vi "Main.vi"(11 "Error In":errorcluster) -> (15 "Error Out":errorcluster)   [LabVIEW 2026]
uses:
  Core/TypeDefs/Enum_Events.ctl
  Core/TypeDefs/Enum_Event_Options.ctl
  Core/TypeDefs/Enum_Queue_Options.ctl
  Core/TypeDefs/Cluster_Queue_Element.ctl
  Core/TypeDefs/Enum_Queues.ctl
  Core/SubVIs/Status_Page/INL-DNL-Status.vi
  Core/Core.lvlib
panel:
  out "Status & Graph":picture
  out "Configuration":picture
  out "Mode Selection":picture
  out "Home":picture
  in  "Tab Sel Buttons":T1(radio)
  in  "Tab Control":T1(tab)
  out "DAC":picture
  out "ADC":picture
  out "Mode Sel Buttons":enum32{"ADC", "DAC"}(radio)
  out "Configuration String":string
  out "Status & Graph String":string
  out "Status":string[][](table)
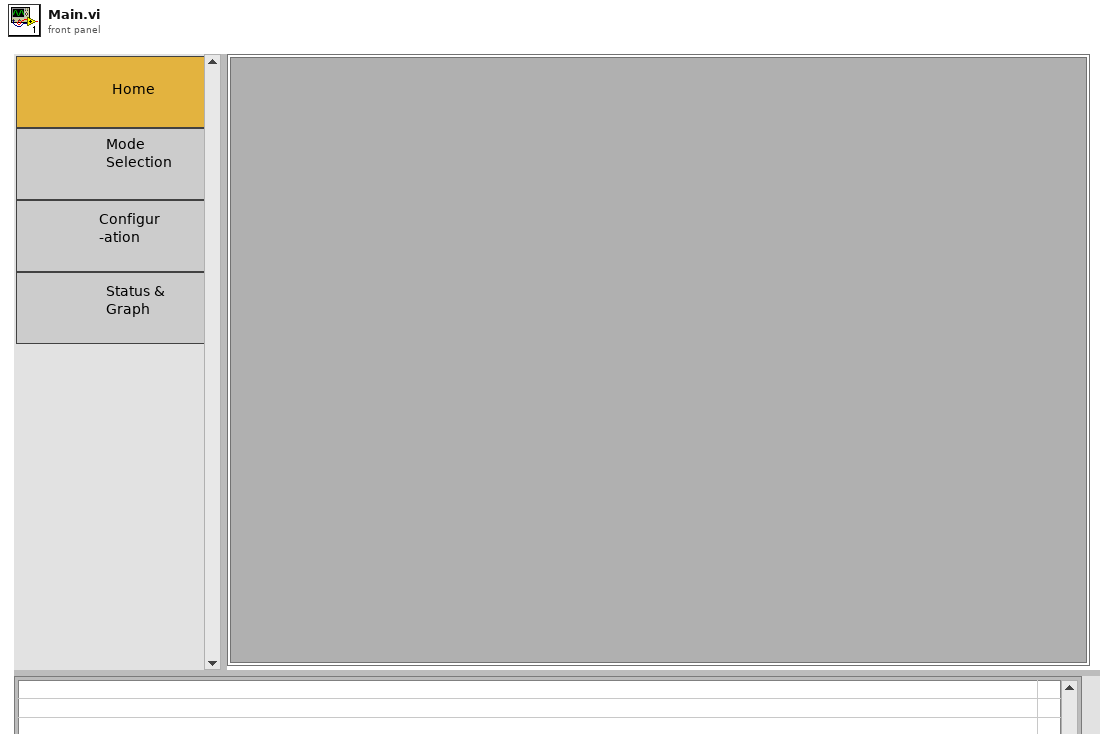
[diagram p1: front panel]
types:
  T1 = enum32{"Home", "Mode Selection", "Configuration", "Status & Graph"}
  T2 = typedef "Core.lvlib/Cluster_Queue_Element.ctl" = cluster{"State":string, "Data":variant}
  T3 = typedef "Core.lvlib/Enum_Queue_Options.ctl" = enum16{"Create", "Enqueue N", "Enstack N", "View Queue", "Dequeue", "Flush", "Flush & Close"}
  T4 = typedef "Core.lvlib/Enum_Queues.ctl" = enum16{"State"}
  T5 = typedef "Core.lvlib/Enum_Event_Options.ctl" = enum16{"Create", "Generate", "Event Ref", "Destroy"}
  T6 = typedef "Core.lvlib/Enum_Events.ctl" = enum16{"Stop All", "Stop SubVI", "Update Object"}
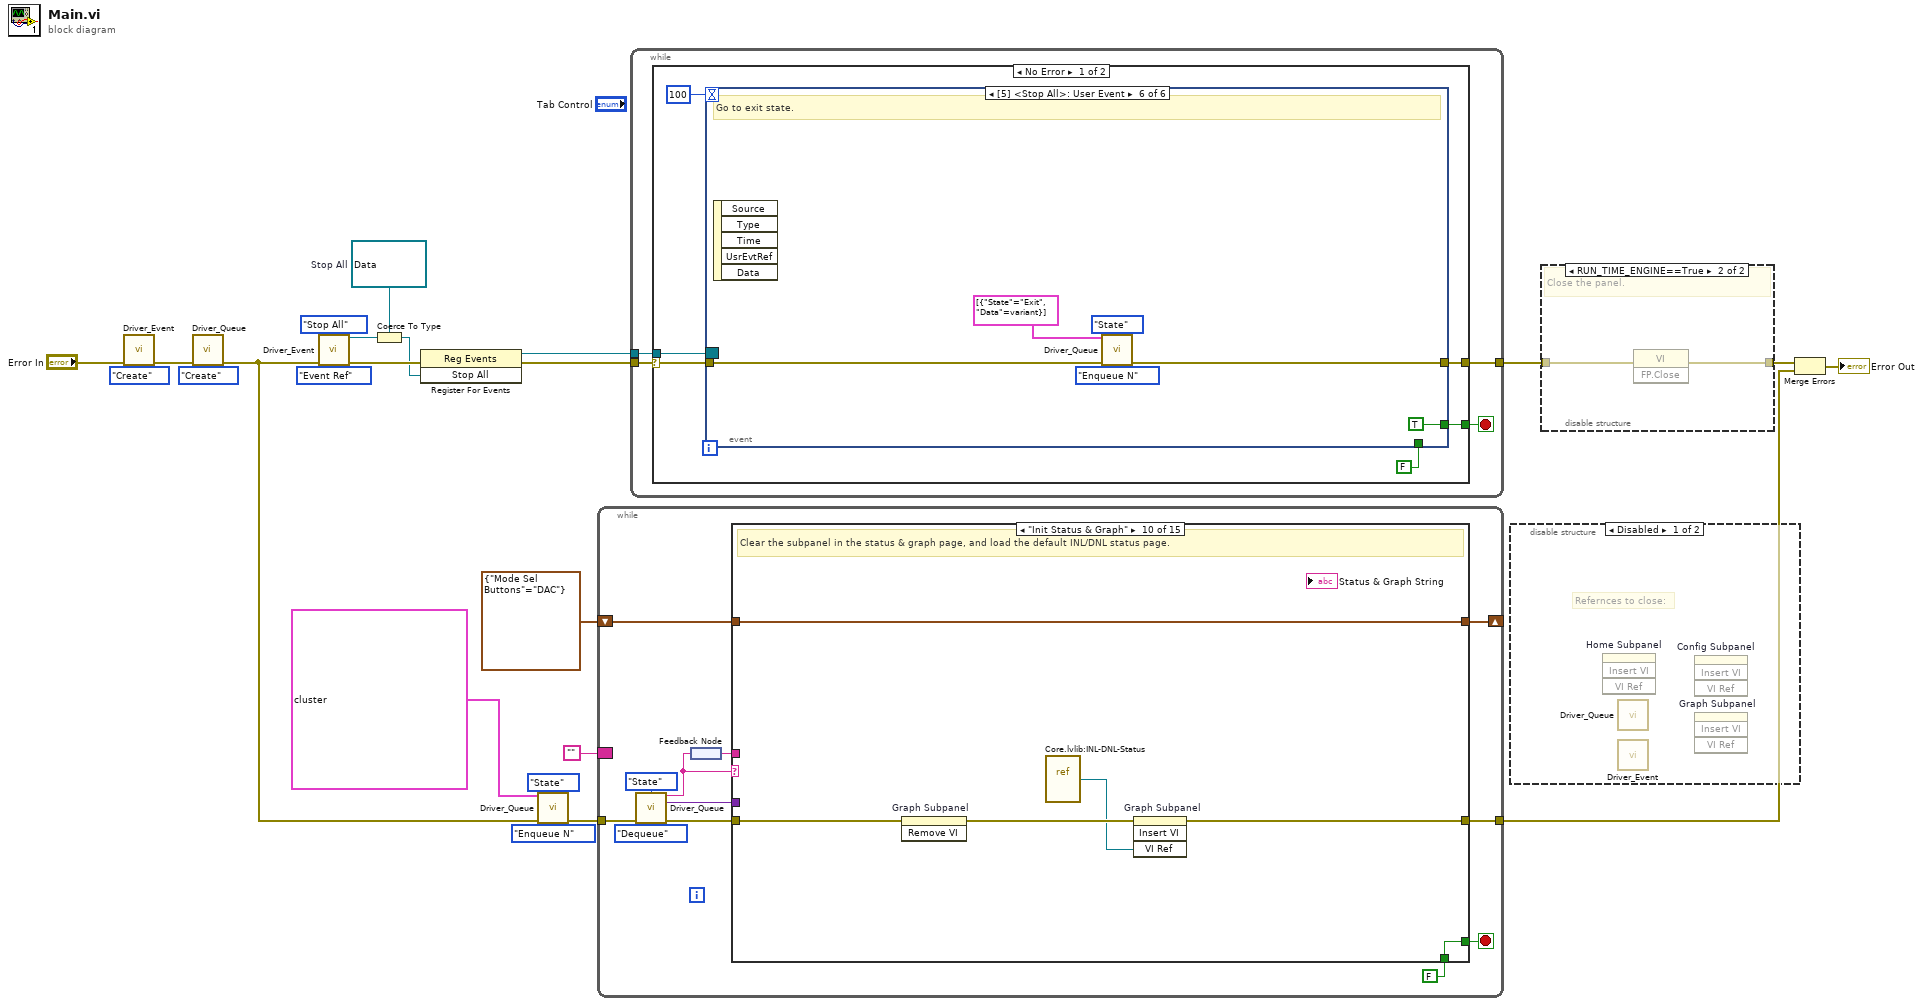
[diagram p0: block diagram]
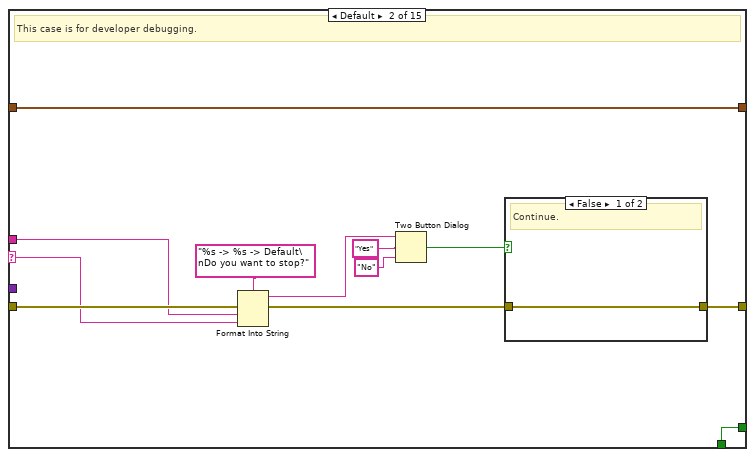
[diagram p5: hidden frame]
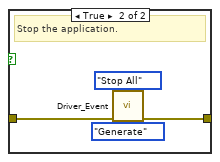
[diagram p6: hidden frame]
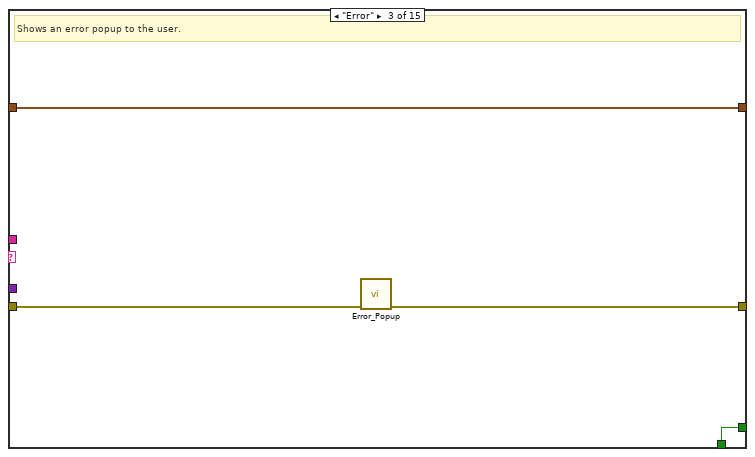
[diagram p7: hidden frame]
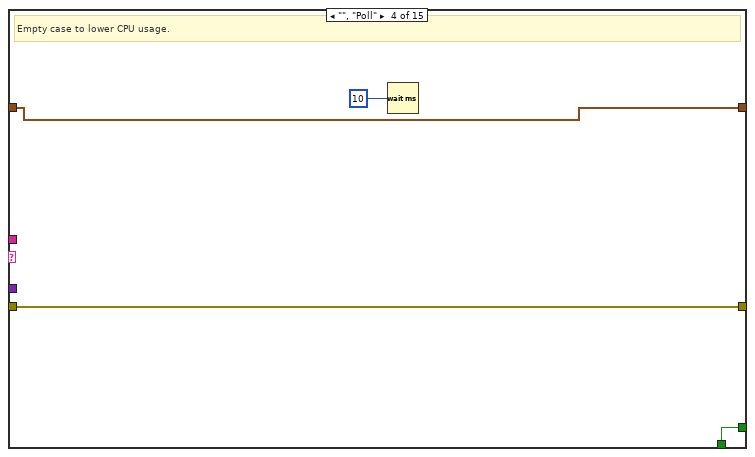
[diagram p8: hidden frame]
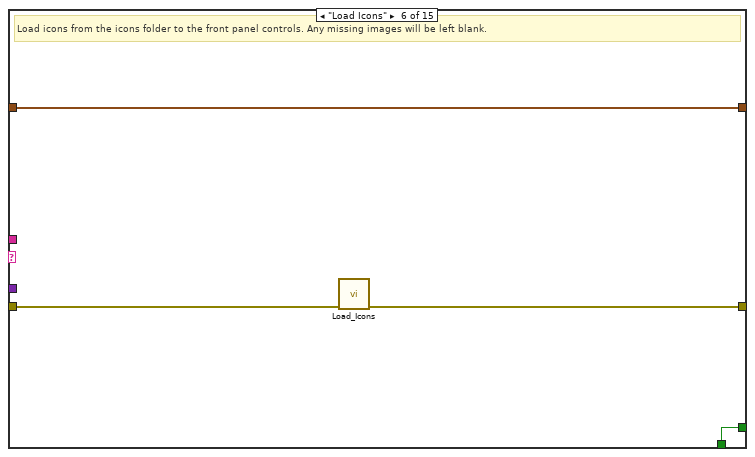
[diagram p10: hidden frame]
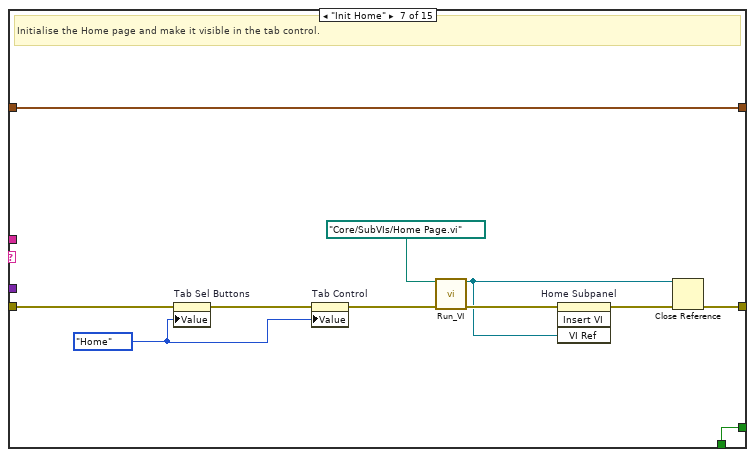
[diagram p11: hidden frame]
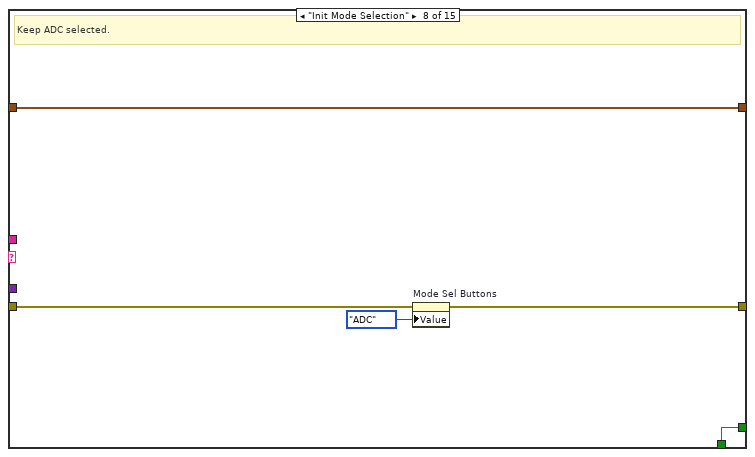
[diagram p12: hidden frame]
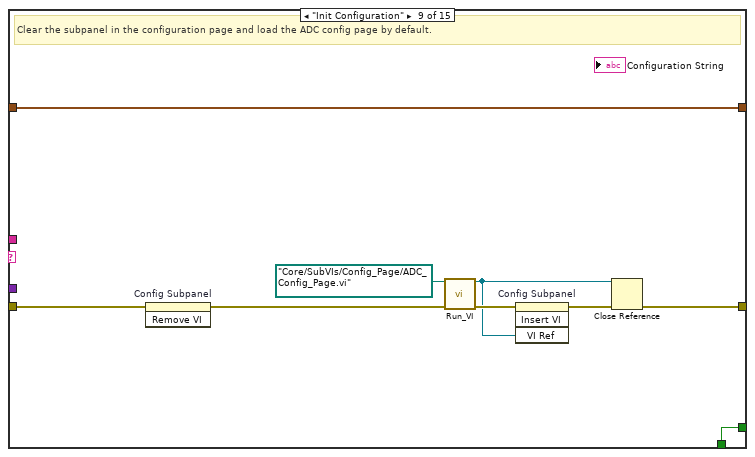
[diagram p13: hidden frame]
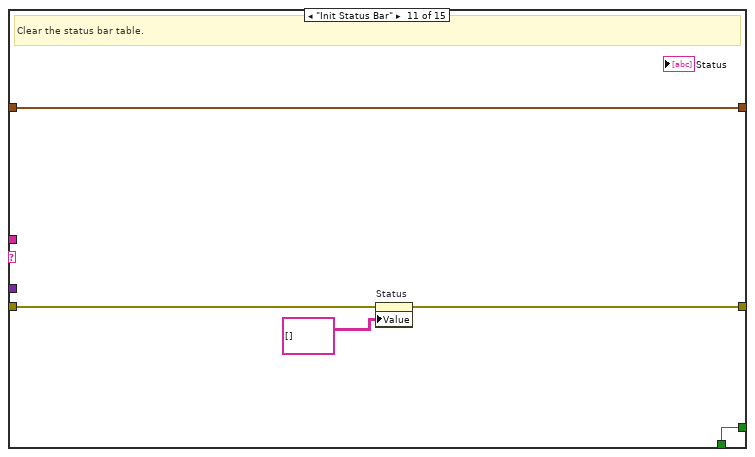
[diagram p14: hidden frame]
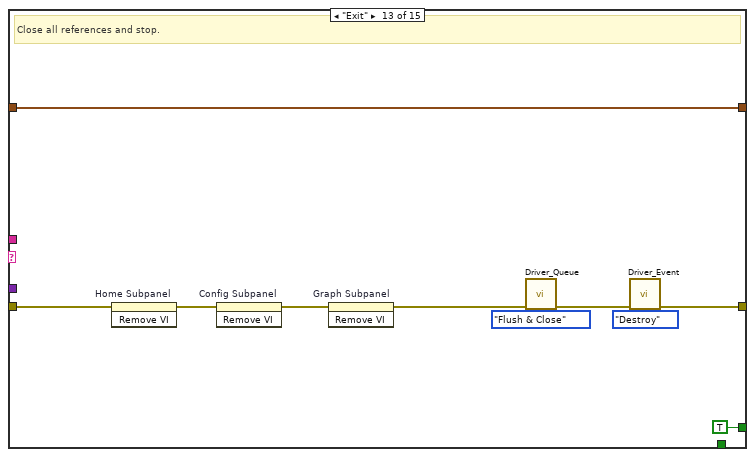
[diagram p16: hidden frame]
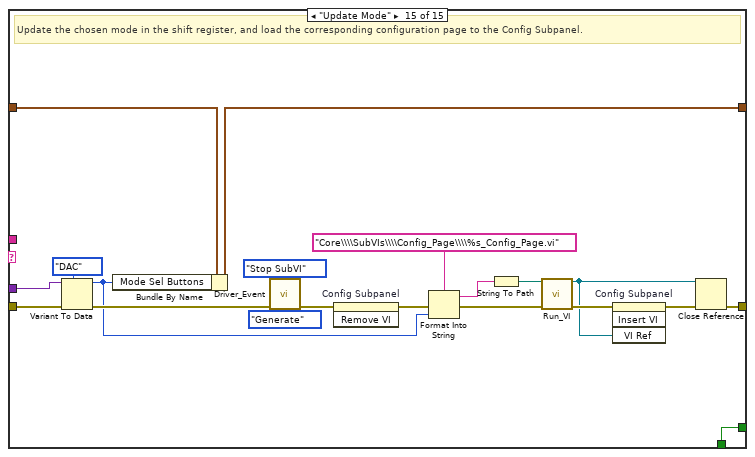
[diagram p18: hidden frame]
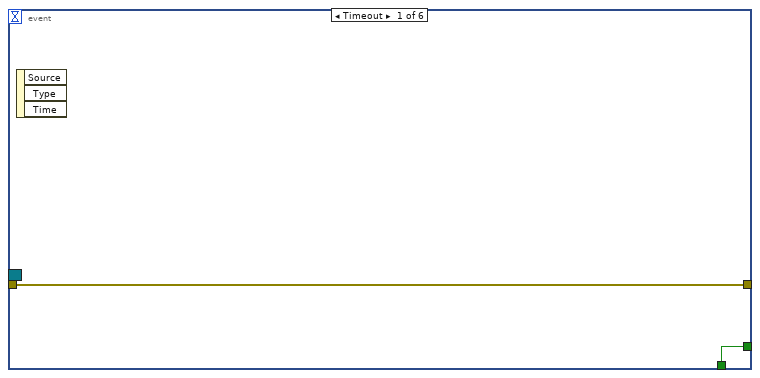
[diagram p19: hidden frame]
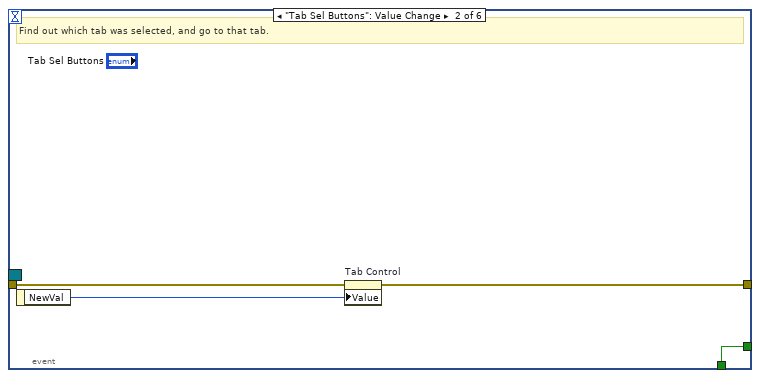
[diagram p20: hidden frame]
diagram:
  w17 = refnum<user-event> refnum  # Stop All
  n1 = call "Driver_Event.vi"("Error In"="Error In", "Event Operation"=Enum_Event_Options."Create") -> ("Error Out"=w22:errorcluster)  [unwired: 12 in, 1 out]
  n2 = call "Driver_Queue.vi"("Error In"=w22, "Queue Operation"=Enum_Queue_Options."Create") -> ("Error Out"=w11:errorcluster)  [unwired: 10 in, 3 out]
  n3 = call "Driver_Event.vi"("Event"=Enum_Events."Stop All", "Error In"=w11, "Event Operation"=Enum_Event_Options."Event Ref") -> ("Event Ref"=w20:refnum<user-event>, "Error Out"=w19:errorcluster)  [unwired: 11 in]
  n4 = Coerce To Type(0:w20, 1:w17) -> (2:w18:refnum<user-event>)
  n5 = register-events(error in=w19, w18) -> (reference out=w12:refnum<event-registration>, error out=w21:errorcluster)  [unwired: 1 in]
  n6 = call "Driver_Queue.vi"("Queue N Elements"=T2[] [{"State"="Load Icons", "Data"=variant}, {"State"="Init Home", "Data"=variant}, {"State"="Init Mode Selection", "Data"=variant}, {"State"="Init Configuration", "Data"=variant}, {"State"="Init Status & Graph", "Data"=variant}, {"State"="Init Status Bar", "Data"=variant}], "Queue"=Enum_Queues."State", "Error In"=w11, "Queue Operation"=Enum_Queue_Options."Enqueue N") -> ("Error Out"=w10:errorcluster)  [unwired: 8 in, 3 out]
  n7 = while {
    tunnel: w10 -> [w32]
    tunnel: [w35] -> w2
    border: "" -> [_]
    shift-right: [w24] -> _
    shift-left: cluster{"Mode Sel Buttons":enum32{"ADC", "DAC"}} {"Mode Sel Buttons"=enum."DAC"} -> [w25]
    stop <- w34 stop-if-true
    n8 = call "Driver_Queue.vi"("Queue"=Enum_Queues."State", "Error In"=w32, "Queue Operation"=Enum_Queue_Options."Dequeue") -> ("State"=w27:string, "Data"=w28:variant, "Error Out"=w31:errorcluster)  [unwired: 9 in, 1 out]
    n9 = feedback-in #1(w27) -> ()
    n10 = feedback #1() -> (w26:string)
    n11 = case shown="\"Init Status & Graph\"" w27 {
      selector: w27 -> [_ w47 _ _ _ _ _ _ _ _ _ _ _ _ _]
      tunnel: [w38 w42 w58 w62 w66 w69 w77 w83 w88 w97 w105 w109 w114 w122 w124] -> w35
      tunnel: [w37 w40 w57 w61 w65 w68 w80 w86 w94 w100 w104 w108 TRUE w121 w137] -> w34
      tunnel: FALSE -> [w37 w40 w57 w61 w65 w68 w80 w86 w94 w100 w104 w108 _ w121 w137]
      tunnel: w31 -> [w38 w50 w59 w62 w66 w70 w74 w84 w95 w101 w106 w109 w119 w122 w142]
      tunnel: w28 -> [_ _ _ _ _ _ _ _ _ _ _ _ _ _ w141]
      tunnel: w26 -> [_ w48 _ _ _ _ _ _ _ _ _ _ _ _ _]
      tunnel: w25 -> [w36 w39 w56 w60 w64 w67 w71 w85 w93 w99 w102 w107 w110 w120 w139]
      tunnel: [w36 w39 w56 w60 w64 w67 w71 w85 w93 w99 w102 w107 w110 w120 w138] -> w24
      frame "/-----General-----/" {
      }
      frame Default {
        # "This case is for developer debugging."
        n12 = Format Into String(format string="%s -> %s -> Default\nDo you want to stop?", error in=w50, w48, w47) -> (resulting string=w46:string, error out=w43:errorcluster)  [unwired: 1 in]
        n13 = Two Button Dialog(message=w46, 1:"No" ("F button name (\"Cancel\")"), 2:"Yes" ("T button name (\"OK\")")) -> (T button?=w41:bool)
        n14 = case shown="False" w41 {
          tunnel: w43 -> [w51 w55]
          tunnel: [w51 w54] -> w42
          frame False {
            # "Continue."
          }
          frame True {
            # "Stop the application."
            n15 = call "Driver_Event.vi"("Event"=Enum_Events."Stop All", "Error In"=w55, "Event Operation"=Enum_Event_Options."Generate") -> ("Error Out"=w54:errorcluster)  [unwired: 11 in, 1 out]
          }
        }
      }
      frame "Error" {
        # "Shows an error popup to the user."
        n16 = call "Error_Popup.vi"("Error In"=w59) -> ("Error Out"=w58:errorcluster)  [unwired: 13 in, 1 out]
      }
      frame "", "Poll" {
        # "Empty case to lower CPU usage."
        n17 = Wait (ms)(milliseconds to wait=u32 10) -> ()  [unwired: 1 out]
      }
      frame "/-----Initialisation-----/" {
      }
      frame "Load Icons" {
        # "Load icons from the icons folder to the front panel controls. Any missing images will be left blank."
        n18 = call "Load_Icons.vi"("Error In"=w70) -> ("Error Out"=w69:errorcluster)  [unwired: 14 in]
      }
      frame "Init Home" {
        w72 = T1."Home" ("Tab Control")
        # "Initialise the Home page and make it visible in the tab control."
        n19 = property on="Tab Sel Buttons" class="RadioBtnsControl (strict)"(error in=w74, "Value"=w72) -> (error out=w73:errorcluster)  [unwired: 1 in, 1 out]
        n20 = property on="Tab Control" class="TabCtl (strict)"(error in=w73, "Value"=w72) -> (error out=w75:errorcluster)  [unwired: 1 in, 1 out]
        n21 = call "Run_VI.vi"("Path"=path "Core/SubVIs/Home Page.vi", "Error In"=w75) -> ("VI Refnum"=w76:refnum<vi>, "Error Out"=w79:errorcluster)  [unwired: 12 in]
        n22 = invoke on="Home Subpanel" class="SubPnl" method="Insert VI"(error in=w79, "VI Ref"=w76) -> (error out=w81:errorcluster)  [unwired: 2 in, 3 out]
        n23 = Close Reference(reference=w76, error in (no error)=w81) -> (error out=w77:errorcluster)
      }
      frame "Init Mode Selection" {
        # "Keep ADC selected."
        n24 = property on="Mode Sel Buttons" class="RadioBtnsControl (strict)"(error in=w84, "Value"=enum32{"ADC", "DAC"}."ADC" ("Mode Sel Buttons")) -> (error out=w83:errorcluster)  [unwired: 1 in, 1 out]
      }
      frame "Init Configuration" {
        # "Clear the subpanel in the configuration page and load the ADC config page by default."
        n25 = invoke on="Config Subpanel" class="SubPnl" method="Remove VI"(error in=w95) -> (error out=w91:errorcluster)  [unwired: 2 in, 2 out]
        n26 = call "Run_VI.vi"("Path"=path "Core/SubVIs/Config_Page/ADC_Config_Page.vi", "Error In"=w91) -> ("VI Refnum"=w87:refnum<vi>, "Error Out"=w92:errorcluster)  [unwired: 12 in]
        n27 = invoke on="Config Subpanel" class="SubPnl" method="Insert VI"(error in=w92, "VI Ref"=w87) -> (error out=w90:errorcluster)  [unwired: 2 in, 3 out]
        n28 = Close Reference(reference=w87, error in (no error)=w90) -> (error out=w88:errorcluster)
      }
      frame "Init Status & Graph" {
        # "Clear the subpanel in the status & graph page, and load the default INL/DNL status page."
        n29 = invoke on="Graph Subpanel" class="SubPnl" method="Remove VI"(error in=w101) -> (error out=w98:errorcluster)  [unwired: 2 in, 2 out]
        n30 = vi-ref "Core.lvlib:INL-DNL-Status.vi"() -> (w96:refnum<vi>)
        n31 = invoke on="Graph Subpanel" class="SubPnl" method="Insert VI"(error in=w98, "VI Ref"=w96) -> (error out=w97:errorcluster)  [unwired: 2 in, 3 out]
      }
      frame "Init Status Bar" {
        # "Clear the status bar table."
        n32 = property on="Status" class="Tbl (strict)"(error in=w106, "Value"=string[][] [] ("Status")) -> (error out=w105:errorcluster)  [unwired: 1 in, 1 out]
      }
      frame "/-----Exit-----/" {
      }
      frame "Exit" {
        # "Close all references and stop."
        n33 = invoke on="Home Subpanel" class="SubPnl" method="Remove VI"(error in=w119) -> (error out=w118:errorcluster)  [unwired: 2 in, 2 out]
        n34 = invoke on="Config Subpanel" class="SubPnl" method="Remove VI"(error in=w118) -> (error out=w117:errorcluster)  [unwired: 2 in, 2 out]
        n35 = invoke on="Graph Subpanel" class="SubPnl" method="Remove VI"(error in=w117) -> (error out=w116:errorcluster)  [unwired: 2 in, 2 out]
        n36 = call "Driver_Queue.vi"("Error In"=w116, "Queue Operation"=Enum_Queue_Options."Flush & Close") -> ("Error Out"=w115:errorcluster)  [unwired: 10 in, 3 out]
        n37 = call "Driver_Event.vi"("Error In"=w115, "Event Operation"=Enum_Event_Options."Destroy") -> ("Error Out"=w114:errorcluster)  [unwired: 12 in, 1 out]
      }
      frame "/-----Mode Selection-----/" {
      }
      frame "Update Mode" {
        # "Update the chosen mode in the shift register, and load the corresponding configuration page to the Config Subpanel."
        n38 = Variant To Data(error in=w142, type=enum32{"ADC", "DAC"}."DAC" ("Mode Sel Buttons"), Variant=w141) -> (data=w131:enum32{"ADC", "DAC"}, error out=w136:errorcluster)
        n39 = Bundle By Name(cluster=w139, "Mode Sel Buttons"=w131) -> (w138:cluster{"Mode Sel Buttons":enum32{"ADC", "DAC"}})
        n40 = call "Driver_Event.vi"("Event"=Enum_Events."Stop SubVI", "Error In"=w136, "Event Operation"=Enum_Event_Options."Generate") -> ("Error Out"=w126:errorcluster)  [unwired: 11 in, 1 out]
        n41 = invoke on="Config Subpanel" class="SubPnl" method="Remove VI"(error in=w126) -> (error out=w125:errorcluster)  [unwired: 2 in, 2 out]
        n42 = Format Into String(format string="Core\\\\SubVIs\\\\Config_Page\\\\%s_Config_Page.vi", error in=w125, w131) -> (resulting string=w130:string, error out=w133:errorcluster)  [unwired: 1 in]
        n43 = String To Path(string=w130) -> (path=w129:path)
        n44 = call "Run_VI.vi"("Path"=w129, "Error In"=w133) -> ("VI Refnum"=w123:refnum<vi>, "Error Out"=w128:errorcluster)  [unwired: 12 in]
        n45 = invoke on="Config Subpanel" class="SubPnl" method="Insert VI"(error in=w128, "VI Ref"=w123) -> (error out=w127:errorcluster)  [unwired: 2 in, 3 out]
        n46 = Close Reference(reference=w123, error in (no error)=w127) -> (error out=w124:errorcluster)
      }
    }
  }
  n47 = while {
    tunnel: w21 -> [w146]
    tunnel: [w145] -> w5
    tunnel: w12 -> [w144]
    stop <- w143 stop-if-true
    n48 = case shown="No Error" w146 {
      selector: w146 -> [w151 w214]
      tunnel: [w150 w213] -> w145
      tunnel: w144 -> [w149 _]
      tunnel: [w148 FALSE] -> w143
      frame No Error {
        n49 = event shown="[5] <Stop All>: User Event" {
          selector: w149 -> [_ _ _ _ _ _]
          dyn-events: _ -> [_ _ _ _ _ _]
          timeout: 100 -> [_ _ _ _ _ _]
          tunnel: w151 -> [w154 w156 w167 w192 w205 w211]
          tunnel: [w154 w158 w160 w186 w204 w210] -> w150
          tunnel: [w153 w157 w165 w188 w203 TRUE] -> w148
          tunnel: FALSE -> [w153 w157 w165 w188 w203 _]
          event Timeout {
            n50 = event-data() -> ()  [unwired: 1 in, 3 out]
          }
          event "Tab Sel Buttons": Value Change {
            # "Find out which tab was selected, and go to that tab."
            n51 = event-data() -> ("NewVal"=w155:T1)  [unwired: 1 in]
            n52 = property on="Tab Control" class="TabCtl (strict)"(error in=w156, "Value"=w155) -> (error out=w158:errorcluster)  [unwired: 1 in, 1 out]
          }
          event "Home", "Mode Selection", "Configuration", "Status & Graph": Mouse Down {
            # "Even if the tab images are clicked, the tab should change."
            n53 = event-data() -> ("CtlRef"=w164:refnum<vi>)  [unwired: 1 in]
            n54 = property class="Pict"(reference=w164, error in=w167) -> (error out=w161:errorcluster, "Label.Text"=w163:string)  [unwired: 1 out]
            n55 = case shown="\"Status & Graph\"" w163 {
              tunnel: [T1."Home" ("Tab Control") T1."Home" ("Tab Control") T1."Mode Selection" ("Tab Control") T1."Configuration" ("Tab Control") T1."Status & Graph" ("Tab Control")] -> w159
              tunnel: [w169 w170 w173 w175 w177] -> w162
              tunnel: w161 -> [w169 w170 w173 w175 w177]
              frame Default {
                # "Set Home as default."
              }
              frame "Home" {
                # "Set the tab to Home."
              }
              frame "Mode Selection" {
                # "Set the tab to Mode Selection."
              }
              frame "Configuration" {
                # "Set the tab to Configuration."
              }
              frame "Status & Graph" {
                # "Set the tab to Status & Graph."
              }
            }
            n56 = property on="Tab Control" class="TabCtl (strict)"(error in=w162, "Value"=w159) -> (error out=w166:errorcluster)  [unwired: 1 in, 1 out]
            n57 = property on="Tab Sel Buttons" class="RadioBtnsControl (strict)"(error in=w166, "Value"=w159) -> (error out=w160:errorcluster)  [unwired: 1 in, 1 out]
          }
          event "ADC", "DAC": Mouse Down {
            # "Highlight the selected device."
            n58 = event-data() -> ("CtlRef"=w193:refnum<vi>)  [unwired: 1 in]
            n59 = property class="Pict"(reference=w193, error in=w192) -> (error out=w190:errorcluster, "Label.Text"=w191:string)  [unwired: 1 out]
            n60 = case shown="\"DAC\"" w191 {
              tunnel: [w195 w197 w199] -> w189
              tunnel: w190 -> [w195 w197 w199]
              tunnel: [enum32{"ADC", "DAC"}."ADC" ("Mode Sel Buttons") enum32{"ADC", "DAC"}."ADC" ("Mode Sel Buttons") enum32{"ADC", "DAC"}."DAC" ("Mode Sel Buttons")] -> w180
              frame Default {
                # "Keep ADC as default."
              }
              frame "ADC" {
                # "Make ADC highlighted."
              }
              frame "DAC" {
                # "Make DAC highlighted."
              }
            }
            n61 = property on="Mode Sel Buttons" class="RadioBtnsControl (strict)"(error in=w189, "Value"=w180) -> (error out=w187:errorcluster)  [unwired: 1 in, 1 out]
            n62 = To Variant(anything=w180) -> (Variant=w181:variant)
            n63 = Bundle By Name(cluster=T2 {"State"="", "Data"=variant} ("Queue Element"), "State"="Update Mode", "Data"=w181) -> (w179:T2)
            n64 = Build Array(w179) -> (w178:T2[])
            n65 = call "Driver_Queue.vi"("Queue N Elements"=w178, "Queue"=Enum_Queues."State", "Error In"=w187, "Queue Operation"=Enum_Queue_Options."Enqueue N") -> ("Error Out"=w186:errorcluster)  [unwired: 8 in, 3 out]
          }
          event Panel Close? {
            # "This stops the application."
            n66 = event-data() -> ()  [unwired: 1 in, 1 out]
            n67 = call "Driver_Event.vi"("Event"=Enum_Events."Stop All", "Error In"=w205, "Event Operation"=Enum_Event_Options."Generate") -> ("Error Out"=w204:errorcluster)  [unwired: 11 in, 1 out]
            n68 = event-data("Discard?"=TRUE) -> ()  [unwired: 1 in, 1 out]
          }
          event User Event {
            # "Go to exit state."
            n69 = event-data() -> ()  [unwired: 1 in, 5 out]
            n70 = call "Driver_Queue.vi"("Queue N Elements"=T2[] [{"State"="Exit", "Data"=variant}], "Queue"=Enum_Queues."State", "Error In"=w211, "Queue Operation"=Enum_Queue_Options."Enqueue N") -> ("Error Out"=w210:errorcluster)  [unwired: 8 in, 3 out]
          }
        }
      }
      frame Error {
        n71 = call "Error_Popup.vi"("Error In"=w214) -> ("Error Out"=w213:errorcluster)  [unwired: 13 in, 1 out]
      }
    }
  }
  n72 = disable-structure shown="Disabled" {
    frame Disabled {
      # "Refernces to close:"
      n73 = invoke on="Home Subpanel" class="SubPnl" method="Insert VI"() -> ()  [unwired: 4 in, 4 out]
      n74 = call "Driver_Queue.vi"() -> ()  [unwired: 12 in, 4 out]
      n75 = call "Driver_Event.vi"() -> ()  [unwired: 14 in, 2 out]
      n76 = invoke on="Config Subpanel" class="SubPnl" method="Insert VI"() -> ()  [unwired: 4 in, 4 out]
      n77 = invoke on="Graph Subpanel" class="SubPnl" method="Insert VI"() -> ()  [unwired: 4 in, 4 out]
    }
    frame Enabled {
    }
  }
  n78 = disable-structure shown="RUN_TIME_ENGINE==True" {
    disable-tunnel: w5 -> [w215 w217]
    disable-tunnel: [w215 w216] -> w4
    frame condition #0 (active) {
      # "Stop normally."
    }
    frame condition #1 {
      # "Close the panel."
      n79 = invoke class="VI" method="FP.Close"(error in=w217) -> (error out=w216:errorcluster)  [unwired: 2 in, 2 out]
    }
  }
  n80 = Merge Errors(w4, w2) -> (→"Error Out":errorcluster)
